vi "Raise or Lower Abort.vi"(8 "error in (no error)":errorcluster, 9 "Sender":string, 10 "New Abort Value":bool, 11 "Guardian in":refnum<class "Guardian.lvclass">) -> (0 "error out":errorcluster, 3 "Guardian out":refnum<class "Guardian.lvclass">)   [LabVIEW 2020, in "TALOS.lvlib" / "Guardian.lvlib" / "Guardian.lvclass"]
uses:
  Guardian.lvclass
  Guardian.lvclass/Guardian.ctl
  Abort Message.ctl
  builds/Actor Framework PPL/Actor Framework.lvlibp/1abvi3w/vi.lib/ActorFramework/Message Enqueuer/Message Priority.ctl
  builds/Actor Framework PPL/Actor Framework.lvlibp/1abvi3w/vi.lib/ActorFramework/Message Enqueuer/Message Enqueuer.lvclass
  Ancestor/Ancestor/Ancestor.lvclass
  Abort Processing actions.ctl
  C:/Users/marco/Documents/GitHub_Lab/TALOS/talos/Ancestor/Ancestor/Ancestor.lvclass
  C:/Users/marco/Documents/GitHub_Lab/TALOS/builds/Actor Framework PPL/Actor Framework.lvlibp/1abvi3w/vi.lib/ActorFramework/Actor/Actor.lvclass
  C:/Users/marco/Documents/GitHub_Lab/TALOS/talos/Guardian/Guardian/Guardian.lvclass
  TALOS.lvlib
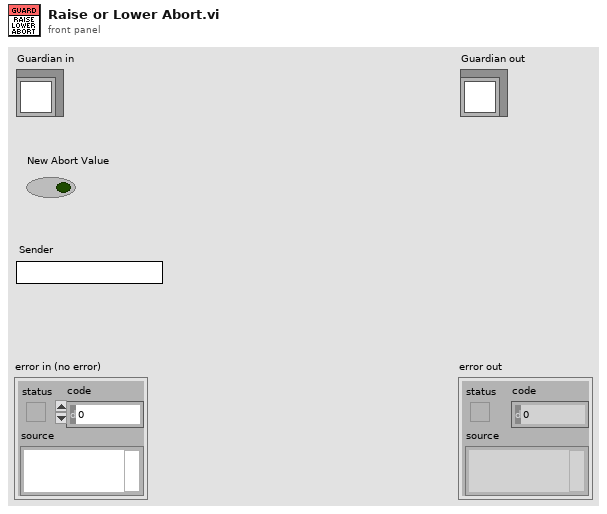
[diagram p1: front panel]
types:
  T1 = typedef "TALOS.lvlib/Guardian.lvlib/Guardian.lvclass/Abort Processing actions.ctl" = enum16{"Propagate locally", "Send to all CIRCUS", "Send to Bearer", "Ignore"}
  T2 = typedef "Actor Framework.lvlibp/Message Enqueuer.lvclass/Message Priority.ctl" = enum16{"Low", "Normal", "High"}
  T3 = typedef "TALOS.lvlib/Guardian.lvlib/Guardian.lvclass/Abort Message.ctl" = cluster{"4b0rt":bool, "Sender":string}
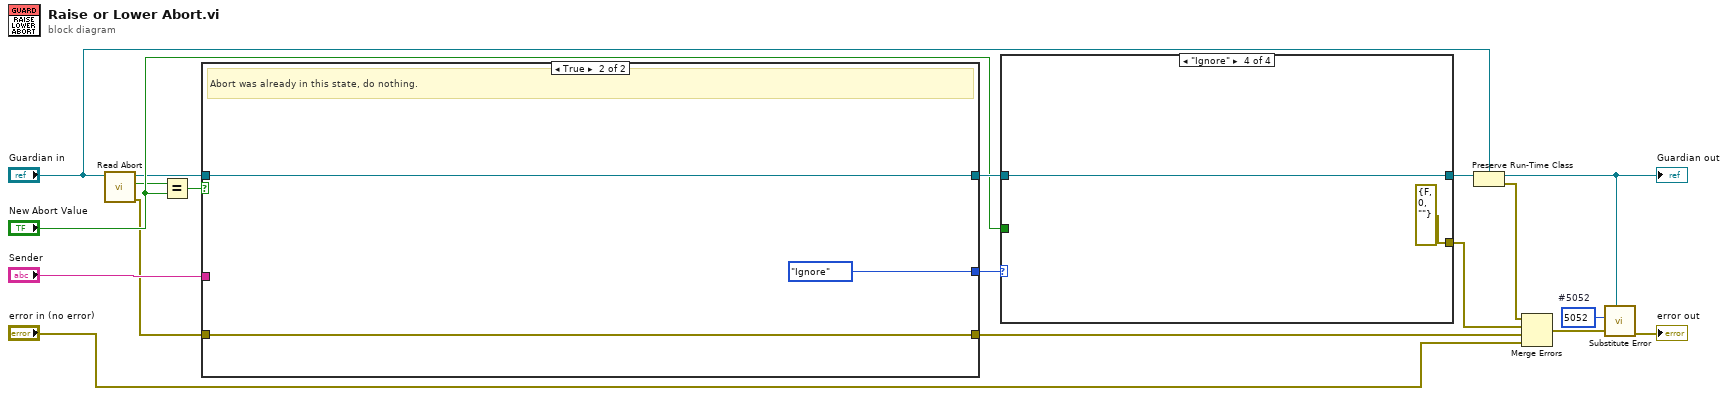
[diagram p0: block diagram]
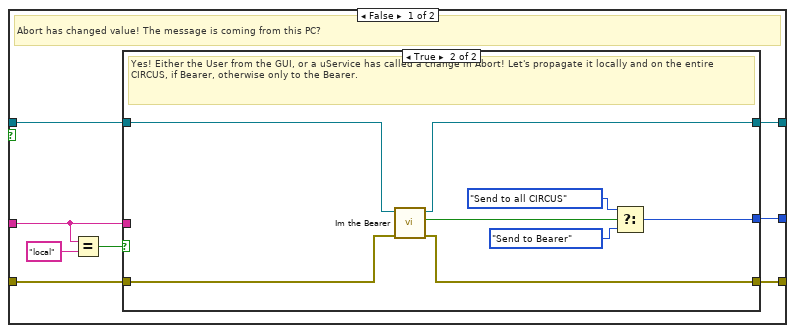
[diagram p2: hidden frame]
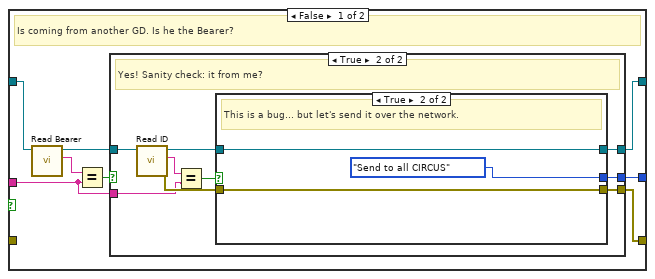
[diagram p3: hidden frame]
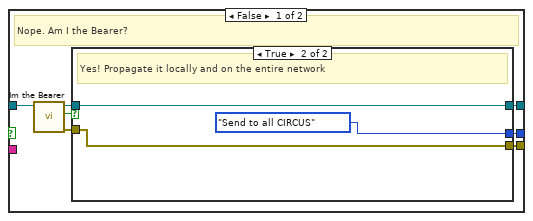
[diagram p4: hidden frame]
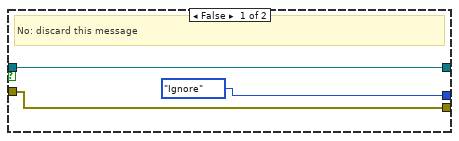
[diagram p5: hidden frame]
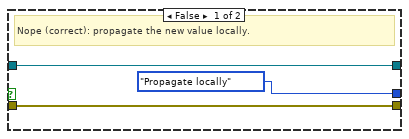
[diagram p6: hidden frame]
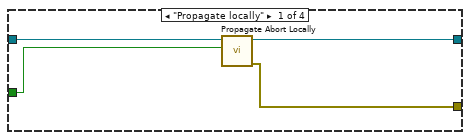
[diagram p7: hidden frame]
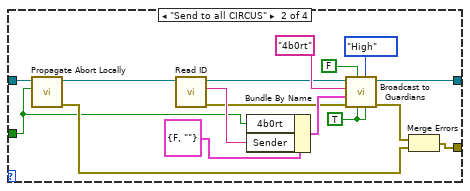
[diagram p8: hidden frame]
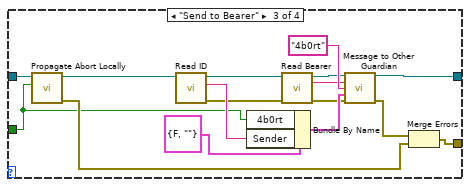
[diagram p9: hidden frame]
diagram:
  w6 = 5052  # #5052
  n1 = call "Read Abort.vi"("Guardian in"="Guardian in") -> ("error out"=w1:errorcluster, "Abort"=w2:bool, "Guardian out"=w4:refnum<class "Guardian.lvclass">)  [unwired: 8 in]
  n2 = Equal?(x=w2, y="New Abort Value") -> (x = y?=w16:bool)
  n3 = case shown="True" w16 {
    tunnel: w4 -> [w25 w73]
    tunnel: [w22 w73] -> w15
    tunnel: w1 -> [w23 w72]
    tunnel: [w20 w72] -> w18
    tunnel: "Sender" -> [w21 _]
    tunnel: [w19 Abort_Processing_actions."Ignore"] -> w13
    frame False {
      # "Abort has changed value! The message is coming from this PC?"
      n4 = Equal?(x=w21, y="local") -> (x = y?=w24:bool)
      n5 = case shown="True" w24 {
        tunnel: w25 -> [w34 w70]
        tunnel: w23 -> [_ w68]
        tunnel: [w29 w67] -> w22
        tunnel: w21 -> [w27 _]
        tunnel: [w30 w69] -> w20
        tunnel: [w28 w64] -> w19
        frame False {
          # "Is coming from another GD. Is he the Bearer?"
          n6 = call "Read Bearer.vi"("Guardian in"=w34) -> ("Bearer"=w33:string, "Guardian out"=w31:refnum<class "Guardian.lvclass">)  [unwired: 8 in, 1 out]
          n7 = Equal?(x=w33, y=w27) -> (x = y?=w32:bool)
          n8 = case shown="True" w32 {
            tunnel: w31 -> [w41 w55]
            tunnel: [w36 w48] -> w30
            tunnel: [w37 w50] -> w29
            tunnel: [w35 w49] -> w28
            tunnel: w27 -> [_ w53]
            frame False {
              # "Nope. Am I the Bearer?"
              n9 = call "Im the Bearer.vi"("Guardian in"=w41) -> ("error out"=w38:errorcluster, "I'm the Bearer"=w40:bool, "Guardian out"=w39:refnum<class "Guardian.lvclass">)  [unwired: 8 in]
              n10 = case shown="True" w40 {
                tunnel: w39 -> [w44 w47]
                tunnel: w38 -> [w43 w46]
                tunnel: [w44 w47] -> w37
                tunnel: [w43 w46] -> w36
                tunnel: [Abort_Processing_actions."Ignore" Abort_Processing_actions."Send to all CIRCUS"] -> w35
                frame False {
                  # "No: discard this message"
                }
                frame True {
                  # "Yes! Propagate it locally and on the entire network"
                }
              }
            }
            frame True {
              # "Yes! Sanity check: it from me?"
              n11 = call "Read ID.vi"("Ancestor in"=w55) -> ("error out"=w56:errorcluster, "ID"=w54:string, "Ancestor out"=w51:refnum<class "Guardian.lvclass">)  [unwired: 8 in]
              n12 = Equal?(x=w54, y=w53) -> (x = y?=w52:bool)
              n13 = case shown="True" w52 {
                tunnel: w51 -> [w59 w62]
                tunnel: [w59 w62] -> w50
                tunnel: [Abort_Processing_actions."Propagate locally" Abort_Processing_actions."Send to all CIRCUS"] -> w49
                tunnel: w56 -> [w57 w60]
                tunnel: [w57 w60] -> w48
                frame False {
                  # "Nope (correct): propagate the new value locally."
                }
                frame True {
                  # "This is a bug... but let's send it over the network."
                }
              }
            }
          }
        }
        frame True {
          # "Yes! Either the User from the GUI, or a uService has called a change in Abort! Let's propagate it locally and on the entire CIRCUS, if Bearer, otherwise only to the Bearer."
          n14 = call "Im the Bearer.vi"("error in (no error)"=w68, "Guardian in"=w70) -> ("error out"=w69:errorcluster, "I'm the Bearer"=w63:bool, "Guardian out"=w67:refnum<class "Guardian.lvclass">)  [unwired: 7 in]
          n15 = Select(t=Abort_Processing_actions."Send to all CIRCUS", s=w63, f=Abort_Processing_actions."Send to Bearer") -> (s? t:f=w64:T1)
        }
      }
    }
    frame True {
      # "Abort was already in this state, do nothing."
    }
  }
  n16 = case shown="\"Ignore\"" w13 {
    tunnel: w15 -> [w76 w84 w100 w111]
    tunnel: [w75 w82 w98 w111] -> w14
    tunnel: "New Abort Value" -> [w74 w81 w97 _]
    tunnel: [w77 w83 w99 errorcluster {"status"=FALSE, "code"=0, "source"=""} ("error IO")] -> w11
    frame "Propagate locally" {
      n17 = call "Propagate Abort Locally.vi"("New Abort Value"=w74, "Guardian in"=w76) -> ("error out"=w77:errorcluster, "Guardian out"=w75:refnum<class "Guardian.lvclass">)  [unwired: 8 in]
    }
    frame "Send to all CIRCUS" {
      w78 = TRUE ("Only active ones?")
      n18 = call "Propagate Abort Locally.vi"("New Abort Value"=w81, "Guardian in"=w84) -> ("error out"=w91:errorcluster, "Guardian out"=w93:refnum<class "Guardian.lvclass">)  [unwired: 8 in]
      n19 = call "Read ID.vi"("Ancestor in"=w93) -> ("error out"=w85:errorcluster, "ID"=w90:string, "Ancestor out"=w86:refnum<class "Guardian.lvclass">)  [unwired: 8 in]
      n20 = Bundle By Name(cluster=T3 {"4b0rt"=FALSE, "Sender"=""} ("4b0rt Message"), "4b0rt"=w81, "Sender"=w90) -> (w88:T3)
      n21 = call "Broadcast to Guardians.vi"("Critical PCs also?"=w78, "Message Priority"=Message_Priority."High", "Only active ones?"=w78, "Local also?"=FALSE, "error in (no error)"=w85, "Data"=w88, "Message"="4b0rt", "Guardian in"=w86) -> ("error out"=w92:errorcluster, "Guardian out"=w82:refnum<class "Guardian.lvclass">)  [unwired: 2 in]
      n22 = Merge Errors(w92, w91) -> (w83:errorcluster)
    }
    frame "Send to Bearer" {
      n23 = call "Propagate Abort Locally.vi"("New Abort Value"=w97, "Guardian in"=w100) -> ("error out"=w107:errorcluster, "Guardian out"=w109:refnum<class "Guardian.lvclass">)  [unwired: 8 in]
      n24 = call "Read ID.vi"("Ancestor in"=w109) -> ("error out"=w101:errorcluster, "ID"=w106:string, "Ancestor out"=w102:refnum<class "Guardian.lvclass">)  [unwired: 8 in]
      n25 = Bundle By Name(cluster=T3 {"4b0rt"=FALSE, "Sender"=""} ("4b0rt Message"), "4b0rt"=w97, "Sender"=w106) -> (w104:T3)
      n26 = call "Read Bearer.vi"("error in (no error)"=w101, "Guardian in"=w102) -> ("error out"=w95:errorcluster, "Bearer"=w94:string, "Guardian out"=w96:refnum<class "Guardian.lvclass">)  [unwired: 7 in]
      n27 = call "Message to Other Guardian.vi"("Guardian in"=w96, "Guardian ID"=w94, "Message"="4b0rt", "Data"=w104, "error in (no error)"=w95) -> ("Guardian out"=w98:refnum<class "Guardian.lvclass">, "error out"=w108:errorcluster)  [unwired: 9 in]
      n28 = Merge Errors(w108, w107) -> (w99:errorcluster)
    }
    frame "Ignore" {
    }
  }
  n29 = Preserve Run-Time Class(object in=w14, 2:"Guardian in") -> (object out=w7:refnum<class "Guardian.lvclass">, error out=w10:errorcluster)  [unwired: 1 in]
  "Guardian out" <- w7
  n30 = Merge Errors(w10, w11, w18, "error in (no error)") -> (w9:errorcluster)
  n31 = call "Substitute Error.vi"("LabVIEW Object"=w7, "error in (no error)"=w9, "Error Code"=w6) -> ("error out"=→"error out":errorcluster)  [unwired: 8 in]
